vi "Update Energized.vi"(6 "Time":dbl, 8 "error in (no error)":errorcluster, 11 "2WayValve in":refnum<class "2WayValveV.lvclass">) -> (0 "error out":errorcluster, 3 "2WayValve out":refnum<class "2WayValveV.lvclass">)   [LabVIEW 2020, in "VolatusGUIElements.lvlib" / "2WayValveV.lvclass"]
uses:
  2WayValveV.lvclass
  2WayValveV.lvclass/2WayValveV.ctl
  lv-vecto/Vecto/Channel DBL/Channel DBL.lvclass/Channel DBL.ctl
  lv-vecto/Vecto/Group DBL/Value by Index.vi
  lv-vecto/Vecto/Channel DBL/Channel DBL.lvclass
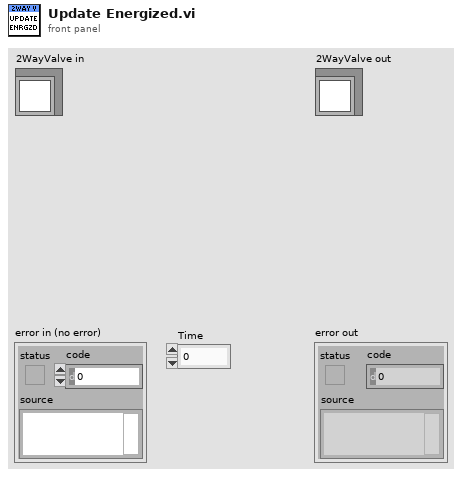
[diagram p1: front panel]
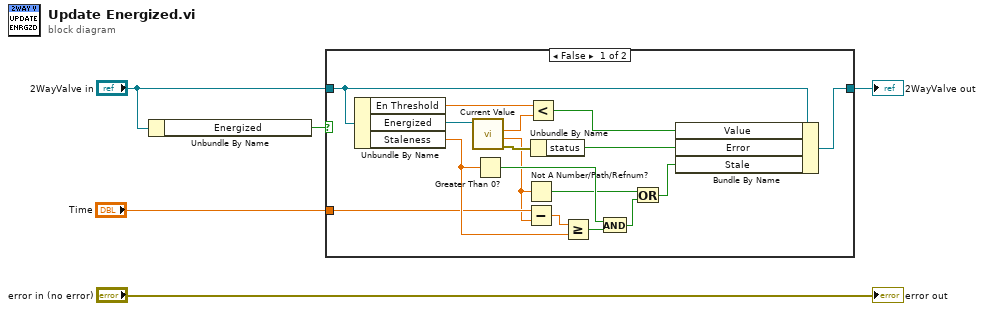
[diagram p0: block diagram]
diagram:
  n1 = Unbundle By Name("2WayValve in") -> ("Energized"=w2:bool)
  n2 = case shown="False" w2 {
    tunnel: [w13 w23] -> w4
    tunnel: "2WayValve in" -> [w14 w23]
    tunnel: "Time" -> [w15 _]
    frame False {
      n3 = Unbundle By Name(w14) -> ("En Threshold"=w8:dbl, "Energized"=w21:refnum<class "Channel DBL.lvclass">, "Staleness"=w18:dbl)
      n4 = call "Current Value.vi"("Channel in"=w21) -> ("error out"=w22:errorcluster, "Timestamp"=w12:dbl, "Scaled"=w7:dbl)  [unwired: 6 in, 2 out]
      n5 = Greater Than 0?(x=w18) -> (x > 0?=w16:bool)
      n6 = Not A Number/Path/Refnum?(number/path/refnum=w12) -> (NaN/Path/Refnum?=w11:bool)
      n7 = Subtract(x=w15, y=w12) -> (x-y=w20:dbl)
      n8 = Less?(x=w8, y=w7) -> (x < y?=w6:bool)
      n9 = Unbundle By Name(w22) -> ("status"=w19:bool)
      n10 = Greater Or Equal?(x=w20, y=w18) -> (x >= y?=w17:bool)
      n11 = And(x=w16, y=w17) -> (x .and. y?=w10:bool)
      n12 = Or(x=w11, y=w10) -> (x .or. y?=w9:bool)
      n13 = Bundle By Name(cluster=w14, "Value"=w6, "Error"=w19, "Stale"=w9) -> (w13:refnum<class "2WayValveV.lvclass">)
    }
    frame True {
      # "Energized Unused"
    }
  }
  "2WayValve out" <- w4
  "error out" <- "error in (no error)"
